vi "World_Load.vi"(11 "error in":errorcluster) -> (4 "Rooms":T1(array[cluster]), 6 "Grid":string[][](array[string]), 15 "error out":errorcluster)   [LabVIEW 2020, in "GH_Level.lvlib"]
doc: "Loads the whole world: reads Resources\\Levels\\world.txt (room grid, depth x column, --- = no room) and every room file with Room_Load. Rooms = all rooms in reading order with ID, Depth, Column and Tiles; Grid = the room IDs as in the file."
uses:
  GH_Level.lvlib
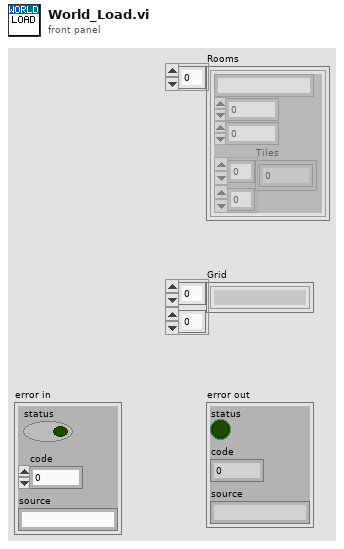
[diagram p1: front panel]
types:
  T1 = cluster{"ID":string, "Depth":i32, "Column":i32, "Tiles":u8[][]}[]
  T2 = cluster{"ID":string, "Depth":i32, "Column":i32, "Tiles":u8[][]}
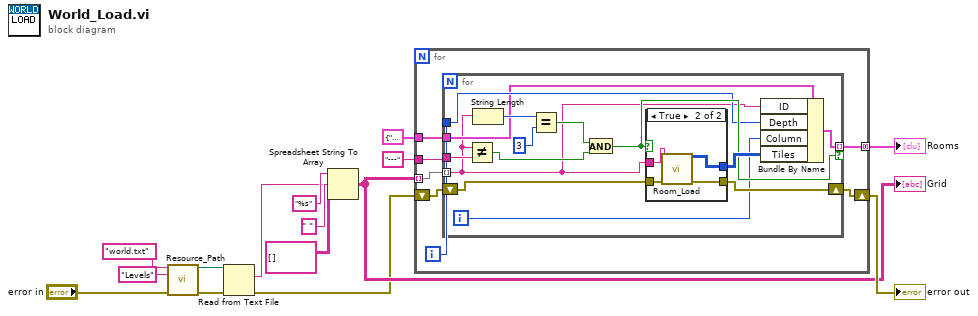
[diagram p0: block diagram]
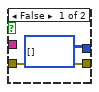
[diagram p2: hidden frame]
diagram:
  n1 = call "Resource_Path.vi"("File name"="world.txt", "Subfolder"="Levels", "error in"="error in") -> ("Path"=w4:path, "error out"=w5:errorcluster)  [unwired: 11 in]
  n2 = Read from Text File(file (use dialog)=w4, error in=w5) -> (text=w6:string, error out=w7:errorcluster)  [unwired: 2 in, 2 out]
  n3 = Spreadsheet String To Array(delimiter (Tab)=" ", format string="%s", spreadsheet string=w6, array type (2D Dbl)=string[][] []) -> (array=w11:string[][])
  "Grid" <- w11
  n4 = for {
    tunnel: "---" -> [w18]
    tunnel: T2 {"ID"="", "Depth"=0, "Column"=0, "Tiles"=[]} -> [w19]
    shift-right: [w21] -> w14
    shift-left: w7 -> [w20]
    tunnel: w11 -> [w17] mode=indexing
    tunnel: [w22] -> w15 mode=concatenating
    i -> [w16]
    n5 = for {
      tunnel: w16 -> [w27]
      tunnel: w18 -> [w25]
      tunnel: w19 -> [w26]
      shift-right: [w29] -> w21
      shift-left: w20 -> [w28]
      tunnel: w17 -> [w24] mode=indexing
      tunnel: [w36] -> w22 mode=indexing if=w34
      i -> [w23]
      n6 = Not Equal?(x=w24, y=w25) -> (x != y?=w33:bool)
      n7 = String Length(string=w24) -> (length=w30:i32)
      n8 = Equal?(x=w30, y=3) -> (x = y?=w32:bool)
      n9 = And(x=w32, y=w33) -> (x .and. y?=w34:bool)
      n10 = case shown="True" w34 {
        tunnel: w28 -> [w37 w40]
        tunnel: w24 -> [_ w39]
        tunnel: [u8[][] [] w41] -> w35
        tunnel: [w37 w42] -> w29
        frame False {
        }
        frame True {
          n11 = call "Room_Load.vi"("Room ID"=w39, "error in"=w40) -> ("Tiles"=w41:u8[][], "error out"=w42:errorcluster)  [unwired: 12 in]
        }
      }
      n12 = Bundle By Name(cluster=w26, "ID"=w24, "Depth"=w27, "Column"=w23, "Tiles"=w35) -> (w36:T2)
    }
  }
  "Rooms" <- w15
  "error out" <- w14
